vi "Update Plot List.vi"(8 "error in (no error)":errorcluster, 10 "曲线列表":T1(array[cluster]) caption="曲线" {"Scale" items=["温度", "湿度"]}, 11 "Data Viewer in":refnum<class "Data Viewer.lvclass">) -> (0 "error out":errorcluster, 3 "Data Viewer out":refnum<class "Data Viewer.lvclass">)   [LabVIEW 2020, in "Data Viewer.lvlib" / "Data Viewer.lvclass"]
uses:
  Data Viewer.lvclass
  Data Viewer.lvclass/Data Viewer.ctl
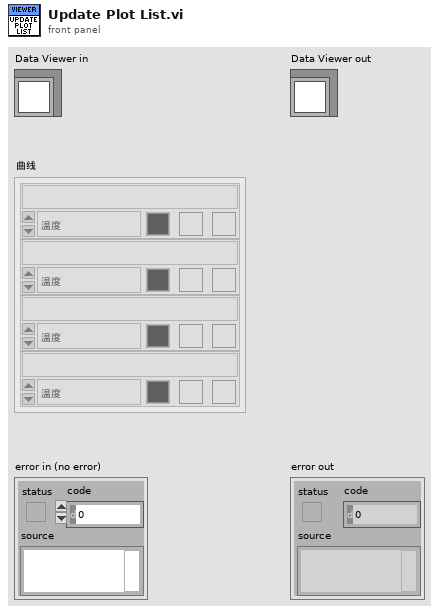
[diagram p1: front panel]
types:
  T1 = cluster{"Name":string, "Scale":u16, "Color":u32, "Visible":bool, "Peak Line":bool}[]
  T2 = typedef "Data Viewer.lvlib/Data Viewer.lvclass/Plot Property--cluster.ctl" = cluster{"Name":string, "Visible":bool, "Color":u32, "Scale Index":i32, "Show Peak Line":bool}
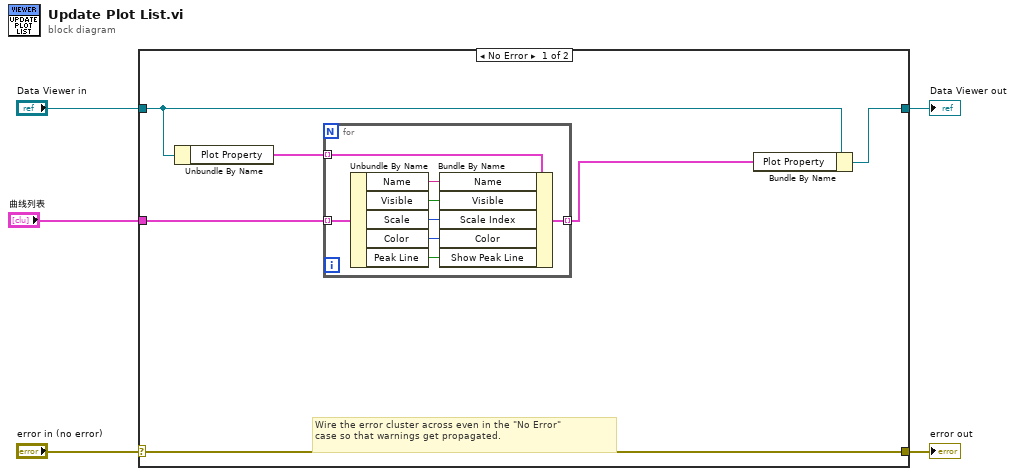
[diagram p0: block diagram]
diagram:
  n1 = case shown="No Error" "error in (no error)" {
    selector: "error in (no error)" -> [w11 w21]
    tunnel: [w11 w21] -> w4
    tunnel: [w7 w20] -> w2
    tunnel: "Data Viewer in" -> [w10 w20]
    tunnel: "曲线列表" -> [w8 _]
    frame No Error {
      # "Wire the error cluster across even in the \"No Error\"\ncase so that warnings get propagated."
      n2 = Unbundle By Name(w10) -> ("Plot Property"=w9:T2[])
      n3 = for {
        tunnel: w9 -> [w19] mode=indexing
        tunnel: w8 -> [w18] mode=indexing
        tunnel: [w12] -> w6 mode=indexing
        n4 = Unbundle By Name(w18) -> ("Name"=w17:string, "Visible"=w16:bool, "Scale"=w15:u16, "Color"=w14:u32, "Peak Line"=w13:bool)
        n5 = Bundle By Name(cluster=w19, "Name"=w17, "Visible"=w16, "Scale Index"=w15, "Color"=w14, "Show Peak Line"=w13) -> (w12:T2)
      }
      n6 = Bundle By Name(cluster=w10, "Plot Property"=w6) -> (w7:refnum<class "Data Viewer.lvclass">)
    }
    frame Error {
    }
  }
  "error out" <- w4
  "Data Viewer out" <- w2
